vi "Module Loop.vi"(8 "error in (no error)":errorcluster, 11 "SoftVar Module in":refnum<class "SoftVar Module.lvclass">) -> (0 "error out":errorcluster, 3 "SoftVar Module out":refnum<class "SoftVar Module.lvclass">)   [LabVIEW 2020, in "Volatus.lvlib" / "SoftVar Module.lvclass"]
uses:
  SoftVar Module.lvclass
  C:/dev/lv20CE/relink/lv-volatus/Volatus/Module/Module.lvclass
  Module/Module.lvclass
  SoftVar Module.lvclass/SoftVar Module.ctl
  messages/CmdAnalog/Class/Msg.lvclass
  C:/dev/lv20CE/relink/lv-protoc/LV-Proto/Message/Message.lvclass
  messages/CmdAnalog/Class/Msg.lvclass/Msg.ctl
  Module/Module.lvclass/Module.ctl
  MessageQ/MessageQ.lvclass/MessageQ.ctl
  messages/CmdAnalog/Data.ctl
  messages/CmdAnalogMultiple/Class/Msg.lvclass
  messages/CmdAnalogMultiple/Class/Msg.lvclass/Msg.ctl
  messages/CmdAnalogMultiple/Data.ctl
  messages/CmdDigital/Class/Msg.lvclass
  messages/CmdDigital/Class/Msg.lvclass/Msg.ctl
  messages/CmdDigital/Data.ctl
  messages/CmdDigitalMultiple/Class/Msg.lvclass
  messages/CmdDigitalMultiple/Class/Msg.lvclass/Msg.ctl
  messages/CmdDigitalMultiple/Data.ctl
  Module/Self Q.vi
  MessageQ/Send.vi
  lv-vecto/Vecto/Group DBL/Update Value by Index.vi
  <vilib>/Utility/error.llb/Error Cluster From Error Code.vi
  messages/CmdAnalog/CmdAnalog.lvlib
  lv-vecto/Vecto/Vecto.lvlib
  messages/CmdDigital/CmdDigital.lvlib
  messages/CmdAnalogMultiple/CmdAnalogMultiple.lvlib
  messages/CmdDigitalMultiple/CmdDigitalMultiple.lvlib
  lv-vecto/Vecto/Group DBL/Group DBL.lvclass
panel:
  in  "Display":bool
  out "Values":T1(array[cluster])
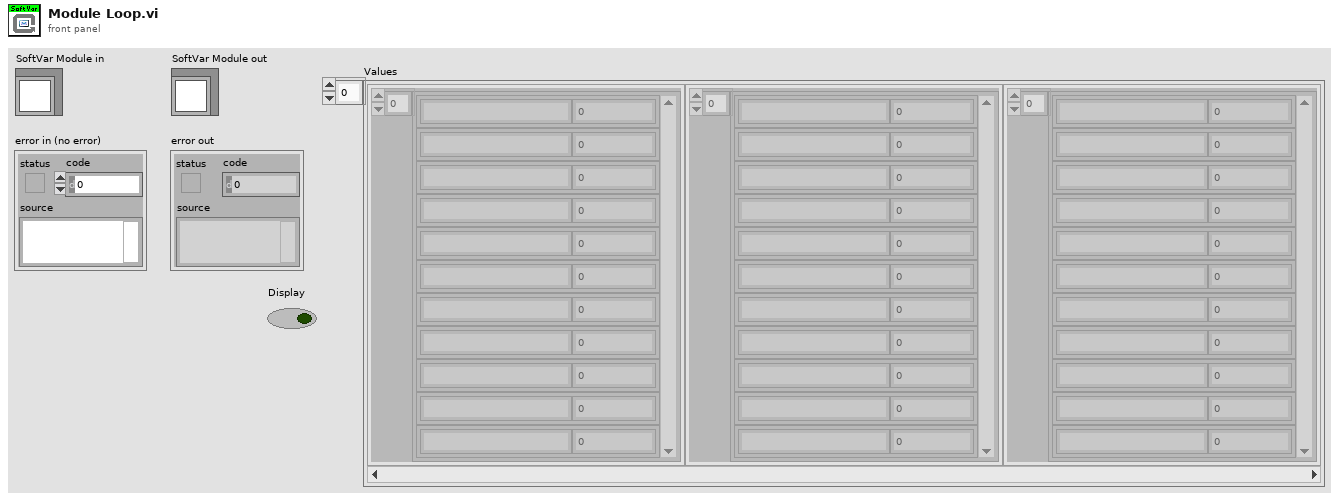
[diagram p1: front panel]
types:
  T1 = cluster{cluster{"Name":string, "Scaled":dbl}[]}[]
  T2 = enum32{"Invalid", "Standard", "Closed", "Hidden", "Minimized", "Maximized"}
  T3 = typedef "CmdAnalog.lvlib/Data.ctl" = cluster{"channel":string, "value":dbl}
  T4 = typedef "CmdAnalogMultiple.lvlib/Data.ctl" = cluster{"values":T3[]}
  T5 = typedef "CmdDigital.lvlib/Data.ctl" = cluster{"channel":string, "value":bool}
  T6 = typedef "CmdDigitalMultiple.lvlib/Data.ctl" = cluster{"values":T5[]}
  T7 = cluster{cluster{"String":string, "Scaled":dbl}[]}
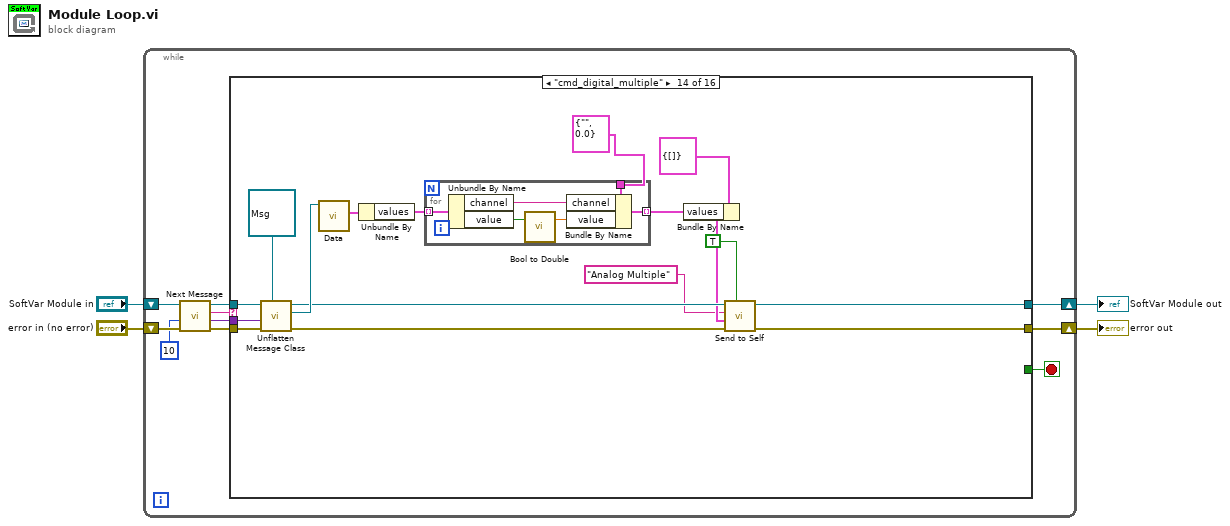
[diagram p0: block diagram]
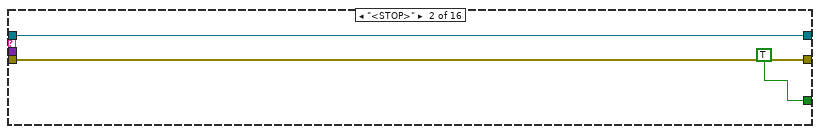
[diagram p3: hidden frame]
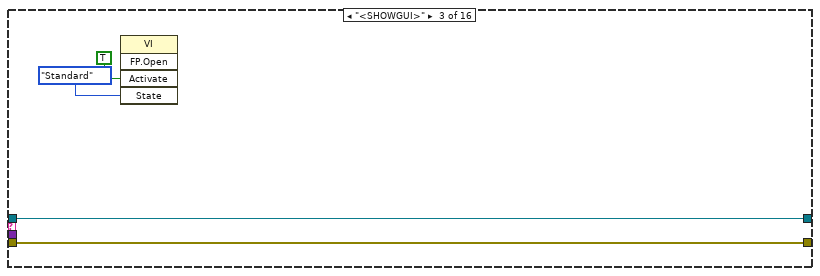
[diagram p4: hidden frame]
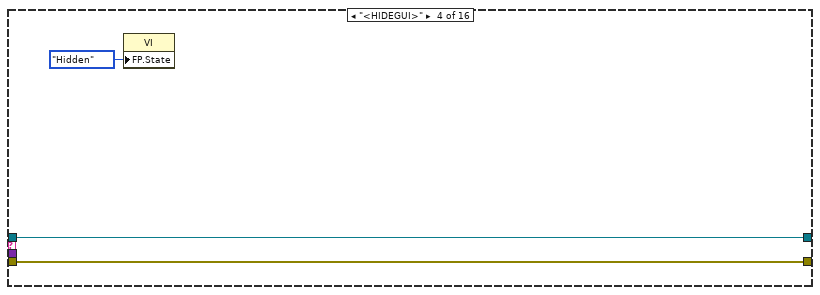
[diagram p5: hidden frame]
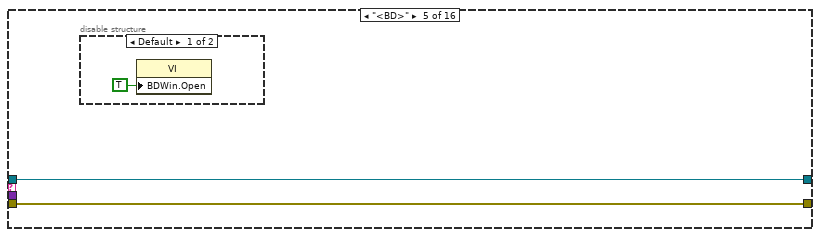
[diagram p6: hidden frame]
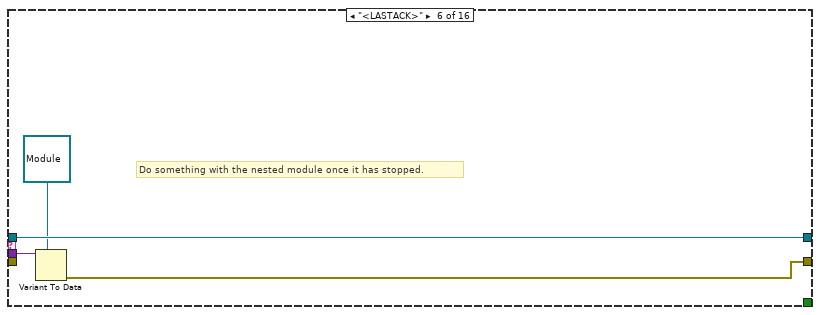
[diagram p8: hidden frame]
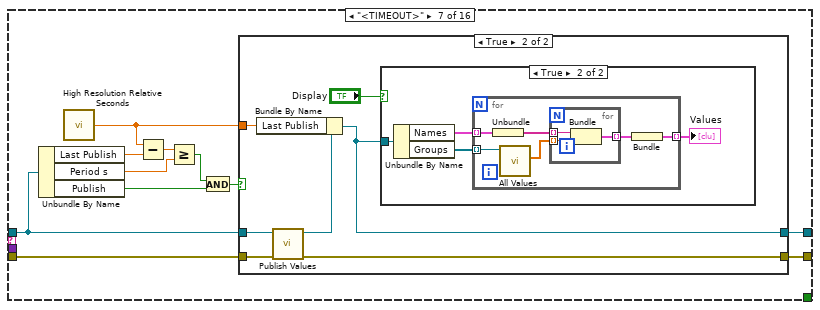
[diagram p9: hidden frame]
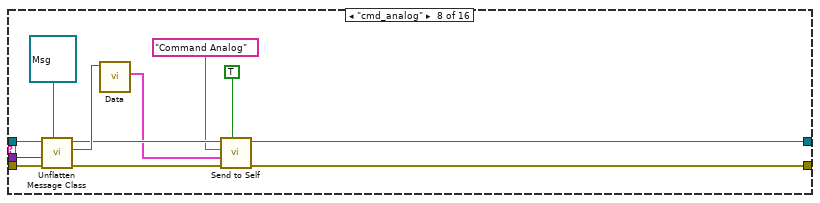
[diagram p12: hidden frame]
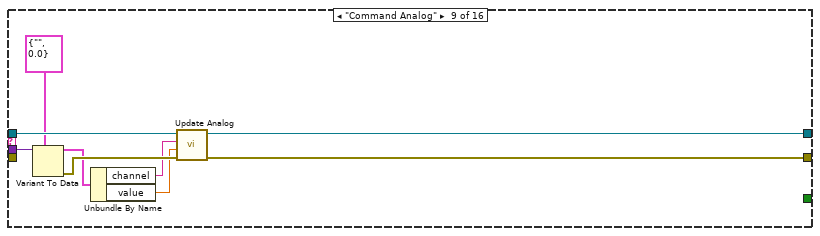
[diagram p13: hidden frame]
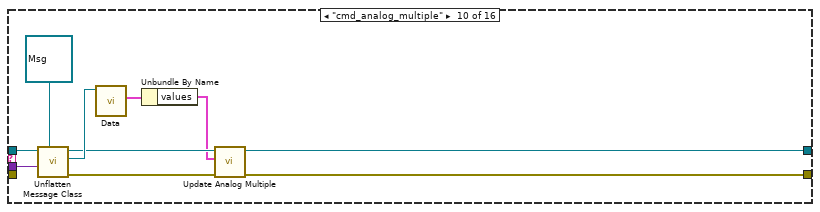
[diagram p14: hidden frame]
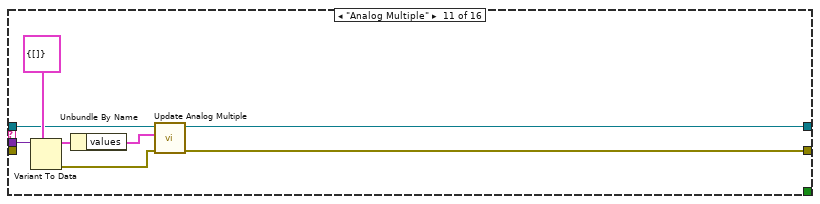
[diagram p15: hidden frame]
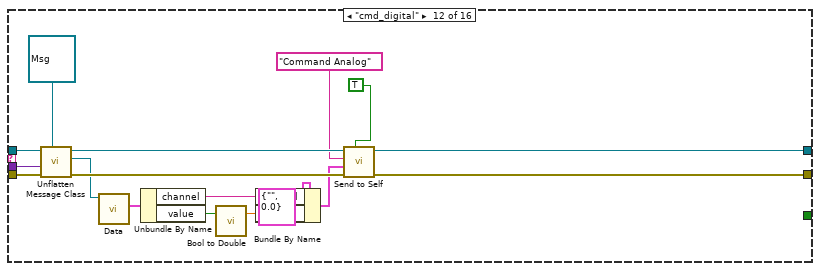
[diagram p16: hidden frame]
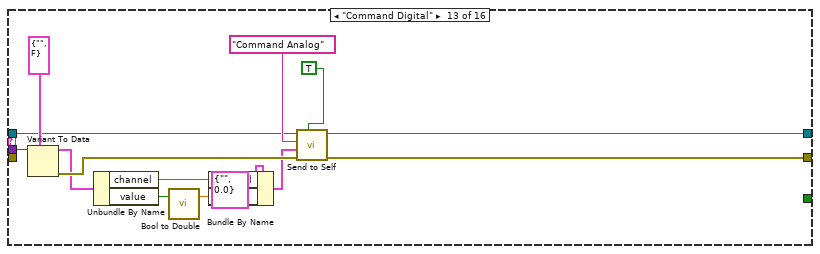
[diagram p17: hidden frame]
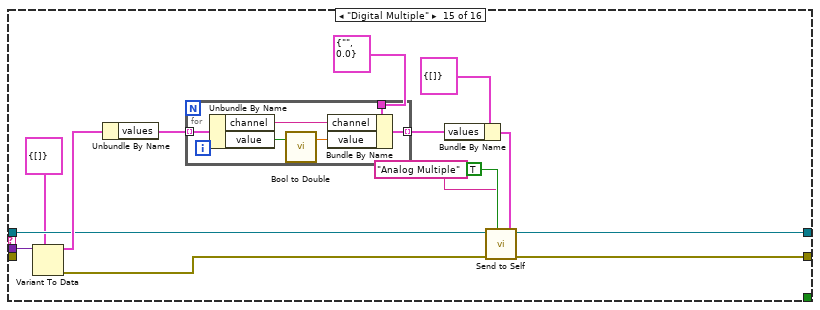
[diagram p18: hidden frame]
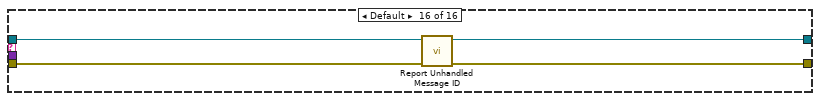
[diagram p19: hidden frame]
diagram:
  n1 = while {
    shift-right: [w9] -> w2
    shift-left: "SoftVar Module in" -> [w14]
    shift-right: [w8] -> w1
    shift-left: "error in (no error)" -> [w13]
    stop <- w7 stop-if-true
    n2 = call "Next Message.vi"("error in (no error)"=w13, "Timeout ms (-1)"=10, "Module in"=w14) -> ("error out"=w12:errorcluster, "Data"=w6:variant, "ID"=w11:string, "Module out"=w10:refnum<class "SoftVar Module.lvclass">)  [unwired: 5 in]
    n3 = case shown="\"cmd_digital_multiple\"" w11 {
      tunnel: w12 -> [w15 w18 w22 w25 w27 _ w41 w70 _ _ _ w115 _ w150 _ w183]
      tunnel: w10 -> [w16 w19 w23 w26 w28 w33 w42 w71 w86 w93 w103 w116 w125 w151 w165 w181]
      tunnel: [w16 w19 w23 w26 w28 w33 w34 w69 w82 w88 w98 w108 w124 w140 w163 w180] -> w9
      tunnel: [w15 w18 w22 w25 w27 w30 w35 w68 w79 w89 w99 w107 w123 w139 w162 w182] -> w8
      tunnel: [_ TRUE _ _ _ _ _ _ _ _ _ _ _ _ _ _] -> w7
      tunnel: w6 -> [_ _ _ _ _ w32 _ w67 w84 w92 w105 w106 w134 w149 w167 _]
      frame "<CLOSE>" {
      }
      frame "<STOP>" {
      }
      frame "<SHOWGUI>" {
        n4 = invoke class="VI" method="FP.Open"("Activate"=TRUE ("Activate?"), "State"=T2."Standard") -> ()  [unwired: 3 in, 5 out]
      }
      frame "<HIDEGUI>" {
        n5 = property class="VI"("FP.State"=T2."Hidden" ("Front Panel Window:State")) -> ()  [unwired: 2 in, 2 out]
      }
      frame "<BD>" {
        n6 = disable-structure shown="Default" {
          frame condition #0 (active) {
            n7 = property class="VI"("BDWin.Open"=TRUE ("Block Diagram Window:Open")) -> ()  [unwired: 2 in, 2 out]
          }
          frame condition #1 {
          }
        }
      }
      frame "<LASTACK>" {
        # "Do something with the nested module once it has stopped."
        n8 = Variant To Data(type=refnum<class "Module.lvclass"> refnum ("Volatus:Module"), Variant=w32) -> (error out=w30:errorcluster)  [unwired: 1 in, 1 out]
      }
      frame "<TIMEOUT>" {
        n9 = Unbundle By Name(w42) -> ("Last Publish"=w44:dbl, "Period s"=w38:dbl, "Publish"=w39:bool)
        n10 = call <vilib>:"High Resolution Relative Seconds.vi"() -> ("relative seconds"=w36:dbl)
        n11 = Subtract(x=w36, y=w44) -> (x-y=w43:dbl)
        n12 = Greater Or Equal?(x=w43, y=w38) -> (x >= y?=w40:bool)
        n13 = And(x=w40, y=w39) -> (x .and. y?=w37:bool)
        n14 = case shown="True" w37 {
          tunnel: w42 -> [w46 w53]
          tunnel: w41 -> [w45 w52]
          tunnel: w36 -> [_ w50]
          tunnel: [w45 w49] -> w35
          tunnel: [w46 w48] -> w34
          frame False {
          }
          frame True {
            n15 = call "Publish Values.vi"("error in (no error)"=w52, "SoftVar Module in"=w53) -> ("error out"=w49:errorcluster, "SoftVar Module out"=w51:refnum<class "SoftVar Module.lvclass">)  [unwired: 8 in]
            n16 = Bundle By Name(cluster=w51, "Last Publish"=w50) -> (w48:refnum<class "SoftVar Module.lvclass">)
            n17 = case shown="False" "Display" {
              tunnel: w48 -> [_ w57]
              frame False {
              }
              frame True {
                n18 = Unbundle By Name(w57) -> ("Names"=w54:cluster{"Names":string[]}[], "Groups"=w56:refnum<class "Group DBL.lvclass">[])
                n19 = for {
                  tunnel: w56 -> [w60] mode=indexing
                  tunnel: [w61] -> w55 mode=indexing
                  tunnel: w54 -> [w59] mode=indexing
                  n20 = Unbundle(w59) -> ("Names"=w58:string[])
                  n21 = call "All Values.vi"("Group in"=w60) -> ("Scaled"=w63:dbl[])  [unwired: 6 in, 4 out]
                  n22 = for {
                    tunnel: w58 -> [w66] mode=indexing
                    tunnel: w63 -> [w65] mode=indexing
                    tunnel: [w64] -> w62 mode=indexing
                    n23 = Bundle("String"=w66, "Scaled"=w65) -> (w64:cluster{"String":string, "Scaled":dbl})  [unwired: 1 in]
                  }
                  n24 = Bundle(w62) -> (w61:T7)  [unwired: 1 in]
                }
                "Values" <- w55
              }
            }
          }
        }
      }
      frame "cmd_analog" {
        n25 = call "Unflatten Message Class.vi"("Message Type"=refnum<class "Msg.lvclass"> refnum ("CmdAnalog.lvlib:Msg.lvclass"), "error in (no error)"=w70, "Data"=w67, "Module in"=w71) -> ("error out"=w75:errorcluster, "Message"=w77:refnum<class "Msg.lvclass">, "Module out"=w76:refnum<class "SoftVar Module.lvclass">)  [unwired: 4 in, 1 out]
        n26 = call "Data.vi"("PB Msg Template in"=w77) -> ("Data"=w74:T3)  [unwired: 8 in, 2 out]
        n27 = call "Send to Self.vi"("High Priority (F)"=TRUE, "error in (no error)"=w75, "Data"=w74, "Message ID"="Command Analog", "Module in"=w76) -> ("error out"=w68:errorcluster, "Module out"=w69:refnum<class "SoftVar Module.lvclass">)  [unwired: 5 in]
      }
      frame "Command Analog" {
        n28 = Variant To Data(type=T3 {"channel"="", "value"=0.0} ("CmdAnalog"), Variant=w84) -> (data=w83:T3, error out=w87:errorcluster)  [unwired: 1 in]
        n29 = Unbundle By Name(w83) -> ("channel"=w81:string, "value"=w80:dbl)
        n30 = call "Update Analog.vi"("error in (no error)"=w87, "Value"=w80, "Channel Name"=w81, "SoftVar Module in"=w86) -> ("error out"=w79:errorcluster, "SoftVar Module out"=w82:refnum<class "SoftVar Module.lvclass">)  [unwired: 6 in]
      }
      frame "cmd_analog_multiple" {
        n31 = call "Unflatten Message Class.vi"("Message Type"=refnum<class "Msg.lvclass"> refnum ("CmdAnalogMultiple.lvlib:Msg.lvclass"), "Data"=w92, "Module in"=w93) -> ("error out"=w97:errorcluster, "Message"=w95:refnum<class "Msg.lvclass">, "Module out"=w91:refnum<class "SoftVar Module.lvclass">)  [unwired: 5 in, 1 out]
        n32 = call "Data.vi"("PB Msg Template in"=w95) -> ("Data"=w94:T4)  [unwired: 8 in, 2 out]
        n33 = Unbundle By Name(w94) -> ("values"=w90:T3[])
        n34 = call "Update Analog Multiple.vi"("error in (no error)"=w97, "Channels"=w90, "SoftVar Module in"=w91) -> ("error out"=w89:errorcluster, "SoftVar Module out"=w88:refnum<class "SoftVar Module.lvclass">)  [unwired: 7 in]
      }
      frame "Analog Multiple" {
        n35 = Variant To Data(type=T4 {"values"=[]} ("CmdAnalogMultiple"), Variant=w105) -> (data=w102:T4, error out=w100:errorcluster)  [unwired: 1 in]
        n36 = Unbundle By Name(w102) -> ("values"=w101:T3[])
        n37 = call "Update Analog Multiple.vi"("error in (no error)"=w100, "Channels"=w101, "SoftVar Module in"=w103) -> ("error out"=w99:errorcluster, "SoftVar Module out"=w98:refnum<class "SoftVar Module.lvclass">)  [unwired: 7 in]
      }
      frame "cmd_digital" {
        n38 = call "Unflatten Message Class.vi"("Message Type"=refnum<class "Msg.lvclass"> refnum ("CmdDigital.lvlib:Msg.lvclass"), "error in (no error)"=w115, "Data"=w106, "Module in"=w116) -> ("error out"=w120:errorcluster, "Message"=w117:refnum<class "Msg.lvclass">, "Module out"=w121:refnum<class "SoftVar Module.lvclass">)  [unwired: 4 in, 1 out]
        n39 = call "Data.vi"("PB Msg Template in"=w117) -> ("Data"=w114:T5)  [unwired: 8 in, 2 out]
        n40 = Unbundle By Name(w114) -> ("channel"=w111:string, "value"=w113:bool)
        n41 = call "Bool to Double.vi"("Bool"=w113) -> ("Double"=w110:dbl)  [unwired: 2 in]
        n42 = Bundle By Name(cluster=T3 {"channel"="", "value"=0.0} ("CmdAnalog"), "channel"=w111, "value"=w110) -> (w109:T3)
        n43 = call "Send to Self.vi"("High Priority (F)"=TRUE, "error in (no error)"=w120, "Data"=w109, "Message ID"="Command Analog", "Module in"=w121) -> ("error out"=w107:errorcluster, "Module out"=w108:refnum<class "SoftVar Module.lvclass">)  [unwired: 5 in]
      }
      frame "Command Digital" {
        n44 = Variant To Data(type=T5 {"channel"="", "value"=FALSE} ("Data"), Variant=w134) -> (data=w126:T5, error out=w136:errorcluster)  [unwired: 1 in]
        n45 = Unbundle By Name(w126) -> ("channel"=w129:string, "value"=w131:bool)
        n46 = call "Bool to Double.vi"("Bool"=w131) -> ("Double"=w128:dbl)  [unwired: 2 in]
        n47 = Bundle By Name(cluster=T3 {"channel"="", "value"=0.0} ("CmdAnalog"), "channel"=w129, "value"=w128) -> (w127:T3)
        n48 = call "Send to Self.vi"("High Priority (F)"=TRUE, "error in (no error)"=w136, "Data"=w127, "Message ID"="Command Analog", "Module in"=w125) -> ("error out"=w123:errorcluster, "Module out"=w124:refnum<class "SoftVar Module.lvclass">)  [unwired: 5 in]
      }
      frame "cmd_digital_multiple" {
        n49 = call "Unflatten Message Class.vi"("Message Type"=refnum<class "Msg.lvclass"> refnum ("CmdDigitalMultiple.lvlib:Msg.lvclass"), "error in (no error)"=w150, "Data"=w149, "Module in"=w151) -> ("error out"=w142:errorcluster, "Message"=w152:refnum<class "Msg.lvclass">, "Module out"=w143:refnum<class "SoftVar Module.lvclass">)  [unwired: 4 in, 1 out]
        n50 = call "Data.vi"("PB Msg Template in"=w152) -> ("Data"=w148:T6)  [unwired: 8 in, 2 out]
        n51 = Unbundle By Name(w148) -> ("values"=w147:T5[])
        n52 = for {
          tunnel: w147 -> [w159] mode=indexing
          tunnel: T3 {"channel"="", "value"=0.0} ("CmdAnalog") -> [w157]
          tunnel: [w154] -> w144 mode=indexing
          n53 = Unbundle By Name(w159) -> ("channel"=w156:string, "value"=w158:bool)
          n54 = call "Bool to Double.vi"("Bool"=w158) -> ("Double"=w155:dbl)  [unwired: 2 in]
          n55 = Bundle By Name(cluster=w157, "channel"=w156, "value"=w155) -> (w154:T3)
        }
        n56 = Bundle By Name(cluster=T4 {"values"=[]} ("Data"), "values"=w144) -> (w138:T4)
        n57 = call "Send to Self.vi"("High Priority (F)"=TRUE, "error in (no error)"=w142, "Data"=w138, "Message ID"="Analog Multiple", "Module in"=w143) -> ("error out"=w139:errorcluster, "Module out"=w140:refnum<class "SoftVar Module.lvclass">)  [unwired: 5 in]
      }
      frame "Digital Multiple" {
        n58 = Variant To Data(type=T6 {"values"=[]} ("CmdDigitalMultiple"), Variant=w167) -> (data=w166:T6, error out=w164:errorcluster)  [unwired: 1 in]
        n59 = Unbundle By Name(w166) -> ("values"=w160:T5[])
        n60 = for {
          tunnel: w160 -> [w179] mode=indexing
          tunnel: T3 {"channel"="", "value"=0.0} ("CmdAnalog") -> [w177]
          tunnel: [w174] -> w171 mode=indexing
          n61 = Unbundle By Name(w179) -> ("channel"=w176:string, "value"=w178:bool)
          n62 = call "Bool to Double.vi"("Bool"=w178) -> ("Double"=w175:dbl)  [unwired: 2 in]
          n63 = Bundle By Name(cluster=w177, "channel"=w176, "value"=w175) -> (w174:T3)
        }
        n64 = Bundle By Name(cluster=T4 {"values"=[]} ("Data"), "values"=w171) -> (w169:T4)
        n65 = call "Send to Self.vi"("High Priority (F)"=TRUE, "error in (no error)"=w164, "Data"=w169, "Message ID"="Analog Multiple", "Module in"=w165) -> ("error out"=w162:errorcluster, "Module out"=w163:refnum<class "SoftVar Module.lvclass">)  [unwired: 5 in]
      }
      frame Default {
        n66 = call "Report Unhandled Message ID.vi"("error in (no error)"=w183, "Module in"=w181) -> ("error out"=w182:errorcluster, "Module out"=w180:refnum<class "SoftVar Module.lvclass">)  [unwired: 8 in]
      }
    }
  }
  "error out" <- w1
  "SoftVar Module out" <- w2
